vi "Test Evaluate Step A Tolerance Edges.vi"(8 "error in":errorcluster) -> (0 "error out":errorcluster)   [LabVIEW 2026]
doc: "Caraya test of Evaluate Step.vi: settling and the tolerance edges 98.0/102.0 in, 97.999/102.001 out for sp 100 tol 2 (EVS-1..5)."
uses:
  <vilib>/addons/_JKI Toolkits/Caraya/classes/Test/Test.lvclass
  <vilib>/addons/_JKI Toolkits/Caraya/classes/Assert/Assert.lvclass
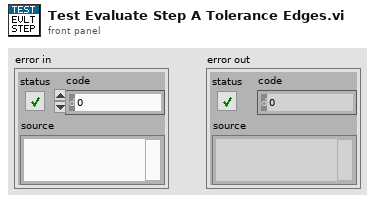
[diagram p1: front panel]
types:
  T1 = cluster{"pressure_bar":dbl, "flow_lpm":dbl, "displacement_mm":dbl, "timestamp_ms":dbl}
  T2 = cluster{"step_no":i32, "step_name":string, "command_type":string, "pressure_sp_bar":dbl, "flow_sp_lpm":dbl, "displacement_sp_mm":dbl, "monitored_io":string, "tolerance_bar":dbl, "dwell_time_ms":i32, "timeout_ms":i32, "expected_result":string}
  T3 = typedef "Step Phase.ctl" = enum16{"Idle", "Settling", "Dwell", "Complete"}
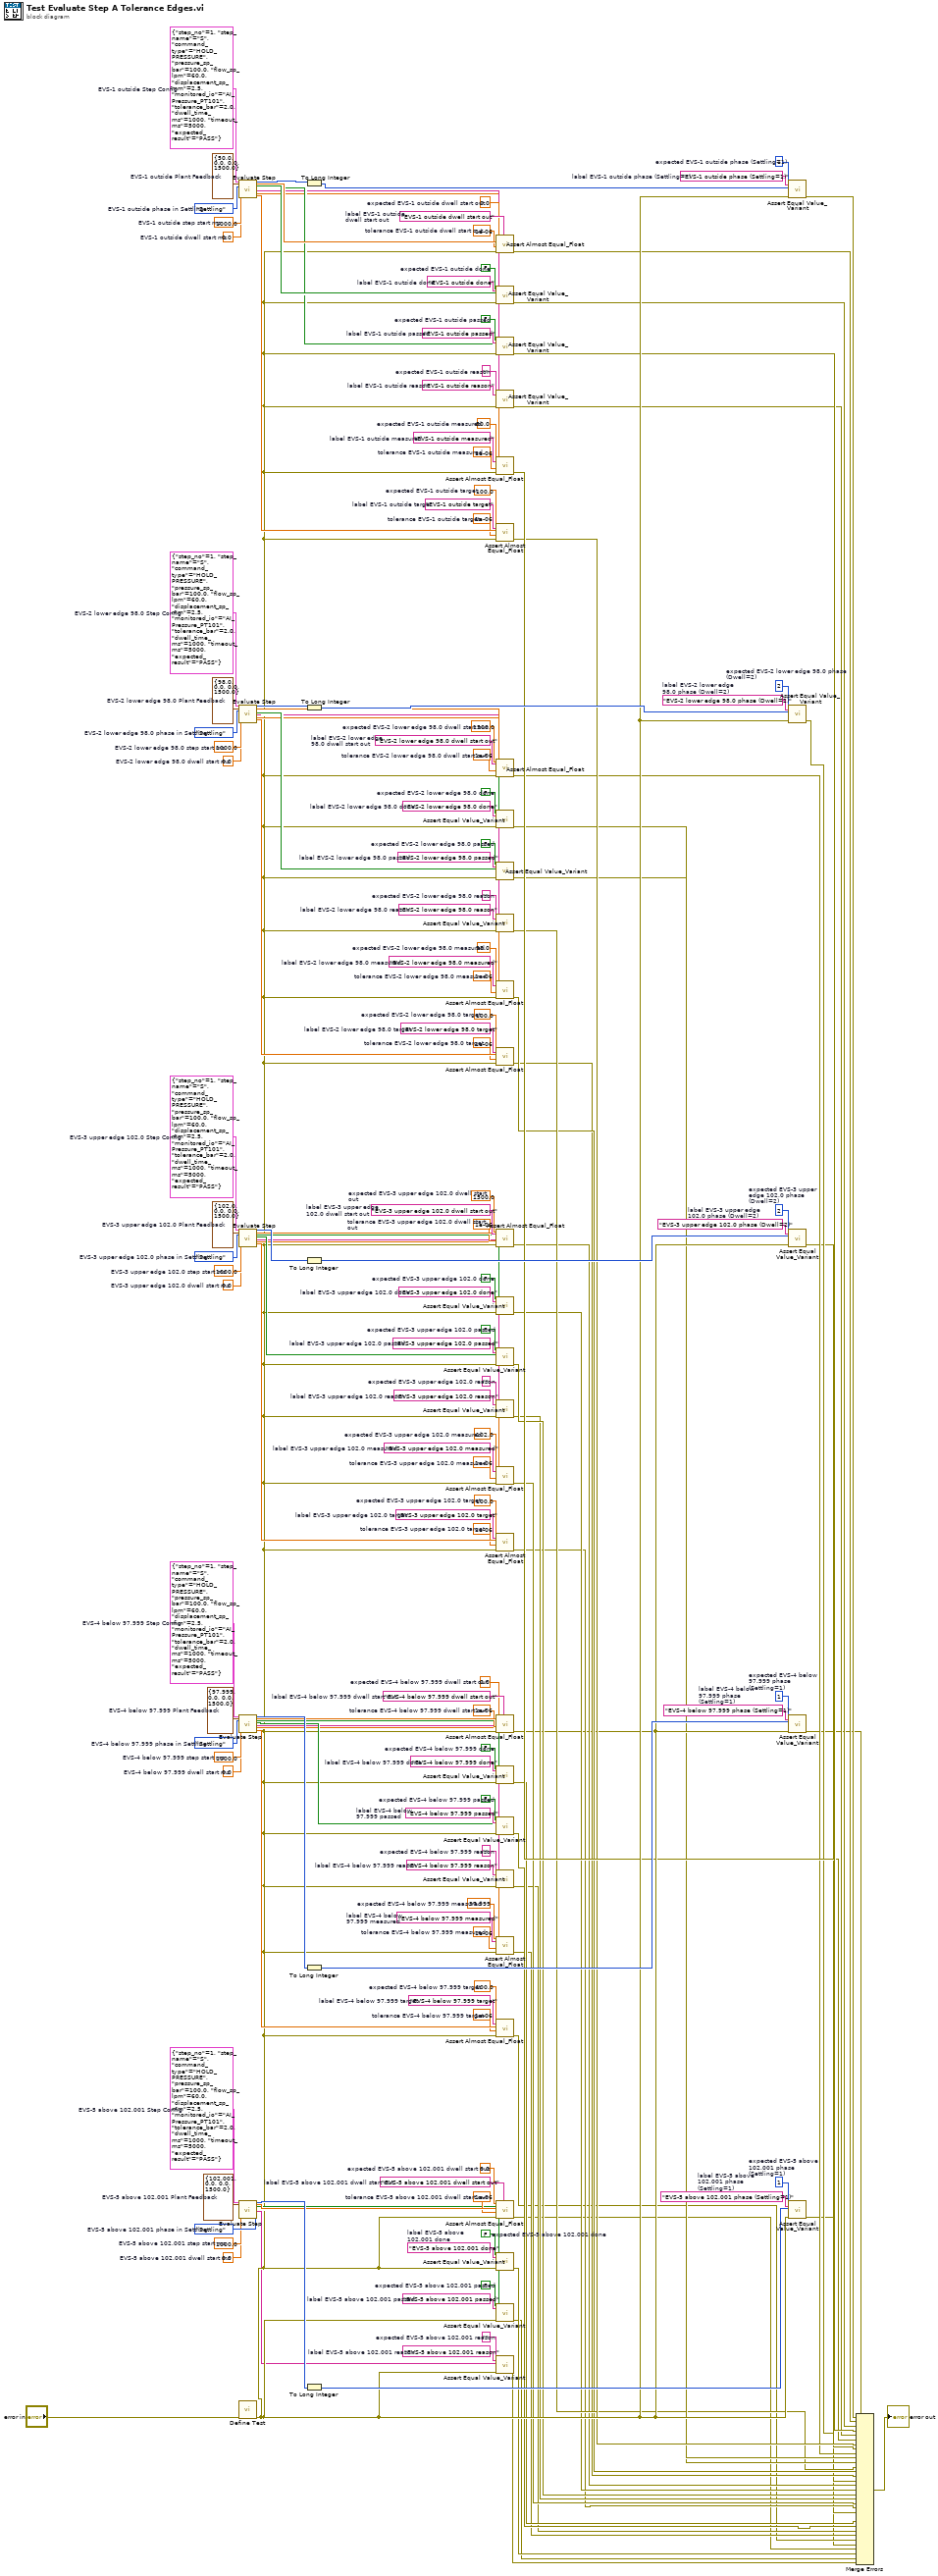
[diagram p0: block diagram]
diagram:
  w38 = "EVS-5 above 102.001 reason"  # label EVS-5 above 102.001 reason
  w36 = ""  # expected EVS-5 above 102.001 reason
  w41 = "EVS-5 above 102.001 passed"  # label EVS-5 above 102.001 passed
  w40 = FALSE  # expected EVS-5 above 102.001 passed
  w44 = "EVS-5 above 102.001 done"  # label EVS-5 above 102.001 done
  w43 = FALSE  # expected EVS-5 above 102.001 done
  w48 = "EVS-5 above 102.001 dwell start out"  # label EVS-5 above 102.001 dwell start out
  w45 = 1e-06  # tolerance EVS-5 above 102.001 dwell start out
  w47 = 0.0  # expected EVS-5 above 102.001 dwell start out
  w51 = "EVS-5 above 102.001 phase (Settling=1)"  # label EVS-5 above 102.001 phase (Settling=1)
  w50 = 1  # expected EVS-5 above 102.001 phase (Settling=1)
  w53 = 0.0  # EVS-5 above 102.001 dwell start ms
  w54 = 1000.0  # EVS-5 above 102.001 step start ms
  w55 = enum16{"Idle", "Settling", "Dwell", "Complete"}."Settling"  # EVS-5 above 102.001 phase in Settling
  w56 = T1 {"pressure_bar"=102.001, "flow_lpm"=0.0, "displacement_mm"=0.0, "timestamp_ms"=1500.0}  # EVS-5 above 102.001 Plant Feedback
  w57 = T2 {"step_no"=1, "step_name"="S", "command_type"="HOLD_PRESSURE", "pressure_sp_bar"=100.0, "flow_sp_lpm"=60.0, "displacement_sp_mm"=2.5, "monitored_io"="AI_Pressure_PT101", "tolerance_bar"=2.0, "dwell_time_ms"=1000, "timeout_ms"=5000, "expected_result"="PASS"}  # EVS-5 above 102.001 Step Config
  w61 = "EVS-4 below 97.999 target"  # label EVS-4 below 97.999 target
  w58 = 1e-06  # tolerance EVS-4 below 97.999 target
  w60 = 100.0  # expected EVS-4 below 97.999 target
  w65 = "EVS-4 below 97.999 measured"  # label EVS-4 below 97.999 measured
  w62 = 1e-06  # tolerance EVS-4 below 97.999 measured
  w64 = 97.999  # expected EVS-4 below 97.999 measured
  w68 = "EVS-4 below 97.999 reason"  # label EVS-4 below 97.999 reason
  w67 = ""  # expected EVS-4 below 97.999 reason
  w71 = "EVS-4 below 97.999 passed"  # label EVS-4 below 97.999 passed
  w70 = FALSE  # expected EVS-4 below 97.999 passed
  w74 = "EVS-4 below 97.999 done"  # label EVS-4 below 97.999 done
  w73 = FALSE  # expected EVS-4 below 97.999 done
  w78 = "EVS-4 below 97.999 dwell start out"  # label EVS-4 below 97.999 dwell start out
  w75 = 1e-06  # tolerance EVS-4 below 97.999 dwell start out
  w77 = 0.0  # expected EVS-4 below 97.999 dwell start out
  w81 = "EVS-4 below 97.999 phase (Settling=1)"  # label EVS-4 below 97.999 phase (Settling=1)
  w80 = 1  # expected EVS-4 below 97.999 phase (Settling=1)
  w83 = 0.0  # EVS-4 below 97.999 dwell start ms
  w84 = 1000.0  # EVS-4 below 97.999 step start ms
  w85 = enum16{"Idle", "Settling", "Dwell", "Complete"}."Settling"  # EVS-4 below 97.999 phase in Settling
  w86 = T1 {"pressure_bar"=97.999, "flow_lpm"=0.0, "displacement_mm"=0.0, "timestamp_ms"=1500.0}  # EVS-4 below 97.999 Plant Feedback
  w87 = T2 {"step_no"=1, "step_name"="S", "command_type"="HOLD_PRESSURE", "pressure_sp_bar"=100.0, "flow_sp_lpm"=60.0, "displacement_sp_mm"=2.5, "monitored_io"="AI_Pressure_PT101", "tolerance_bar"=2.0, "dwell_time_ms"=1000, "timeout_ms"=5000, "expected_result"="PASS"}  # EVS-4 below 97.999 Step Config
  w91 = "EVS-3 upper edge 102.0 target"  # label EVS-3 upper edge 102.0 target
  w88 = 1e-06  # tolerance EVS-3 upper edge 102.0 target
  w90 = 100.0  # expected EVS-3 upper edge 102.0 target
  w95 = "EVS-3 upper edge 102.0 measured"  # label EVS-3 upper edge 102.0 measured
  w92 = 1e-06  # tolerance EVS-3 upper edge 102.0 measured
  w94 = 102.0  # expected EVS-3 upper edge 102.0 measured
  w98 = "EVS-3 upper edge 102.0 reason"  # label EVS-3 upper edge 102.0 reason
  w97 = ""  # expected EVS-3 upper edge 102.0 reason
  w101 = "EVS-3 upper edge 102.0 passed"  # label EVS-3 upper edge 102.0 passed
  w100 = FALSE  # expected EVS-3 upper edge 102.0 passed
  w104 = "EVS-3 upper edge 102.0 done"  # label EVS-3 upper edge 102.0 done
  w103 = FALSE  # expected EVS-3 upper edge 102.0 done
  w108 = "EVS-3 upper edge 102.0 dwell start out"  # label EVS-3 upper edge 102.0 dwell start out
  w105 = 1e-06  # tolerance EVS-3 upper edge 102.0 dwell start out
  w107 = 1500.0  # expected EVS-3 upper edge 102.0 dwell start out
  w111 = "EVS-3 upper edge 102.0 phase (Dwell=2)"  # label EVS-3 upper edge 102.0 phase (Dwell=2)
  w110 = 2  # expected EVS-3 upper edge 102.0 phase (Dwell=2)
  w113 = 0.0  # EVS-3 upper edge 102.0 dwell start ms
  w114 = 1000.0  # EVS-3 upper edge 102.0 step start ms
  w115 = enum16{"Idle", "Settling", "Dwell", "Complete"}."Settling"  # EVS-3 upper edge 102.0 phase in Settling
  w116 = T1 {"pressure_bar"=102.0, "flow_lpm"=0.0, "displacement_mm"=0.0, "timestamp_ms"=1500.0}  # EVS-3 upper edge 102.0 Plant Feedback
  w117 = T2 {"step_no"=1, "step_name"="S", "command_type"="HOLD_PRESSURE", "pressure_sp_bar"=100.0, "flow_sp_lpm"=60.0, "displacement_sp_mm"=2.5, "monitored_io"="AI_Pressure_PT101", "tolerance_bar"=2.0, "dwell_time_ms"=1000, "timeout_ms"=5000, "expected_result"="PASS"}  # EVS-3 upper edge 102.0 Step Config
  w121 = "EVS-2 lower edge 98.0 target"  # label EVS-2 lower edge 98.0 target
  w118 = 1e-06  # tolerance EVS-2 lower edge 98.0 target
  w120 = 100.0  # expected EVS-2 lower edge 98.0 target
  w125 = "EVS-2 lower edge 98.0 measured"  # label EVS-2 lower edge 98.0 measured
  w122 = 1e-06  # tolerance EVS-2 lower edge 98.0 measured
  w124 = 98.0  # expected EVS-2 lower edge 98.0 measured
  w128 = "EVS-2 lower edge 98.0 reason"  # label EVS-2 lower edge 98.0 reason
  w127 = ""  # expected EVS-2 lower edge 98.0 reason
  w131 = "EVS-2 lower edge 98.0 passed"  # label EVS-2 lower edge 98.0 passed
  w130 = FALSE  # expected EVS-2 lower edge 98.0 passed
  w134 = "EVS-2 lower edge 98.0 done"  # label EVS-2 lower edge 98.0 done
  w133 = FALSE  # expected EVS-2 lower edge 98.0 done
  w138 = "EVS-2 lower edge 98.0 dwell start out"  # label EVS-2 lower edge 98.0 dwell start out
  w135 = 1e-06  # tolerance EVS-2 lower edge 98.0 dwell start out
  w137 = 1500.0  # expected EVS-2 lower edge 98.0 dwell start out
  w141 = "EVS-2 lower edge 98.0 phase (Dwell=2)"  # label EVS-2 lower edge 98.0 phase (Dwell=2)
  w140 = 2  # expected EVS-2 lower edge 98.0 phase (Dwell=2)
  w143 = 0.0  # EVS-2 lower edge 98.0 dwell start ms
  w144 = 1000.0  # EVS-2 lower edge 98.0 step start ms
  w145 = enum16{"Idle", "Settling", "Dwell", "Complete"}."Settling"  # EVS-2 lower edge 98.0 phase in Settling
  w146 = T1 {"pressure_bar"=98.0, "flow_lpm"=0.0, "displacement_mm"=0.0, "timestamp_ms"=1500.0}  # EVS-2 lower edge 98.0 Plant Feedback
  w147 = T2 {"step_no"=1, "step_name"="S", "command_type"="HOLD_PRESSURE", "pressure_sp_bar"=100.0, "flow_sp_lpm"=60.0, "displacement_sp_mm"=2.5, "monitored_io"="AI_Pressure_PT101", "tolerance_bar"=2.0, "dwell_time_ms"=1000, "timeout_ms"=5000, "expected_result"="PASS"}  # EVS-2 lower edge 98.0 Step Config
  w151 = "EVS-1 outside target"  # label EVS-1 outside target
  w148 = 1e-06  # tolerance EVS-1 outside target
  w150 = 100.0  # expected EVS-1 outside target
  w155 = "EVS-1 outside measured"  # label EVS-1 outside measured
  w152 = 1e-06  # tolerance EVS-1 outside measured
  w154 = 50.0  # expected EVS-1 outside measured
  w158 = "EVS-1 outside reason"  # label EVS-1 outside reason
  w157 = ""  # expected EVS-1 outside reason
  w161 = "EVS-1 outside passed"  # label EVS-1 outside passed
  w160 = FALSE  # expected EVS-1 outside passed
  w164 = "EVS-1 outside done"  # label EVS-1 outside done
  w163 = FALSE  # expected EVS-1 outside done
  w168 = "EVS-1 outside dwell start out"  # label EVS-1 outside dwell start out
  w165 = 1e-06  # tolerance EVS-1 outside dwell start out
  w167 = 0.0  # expected EVS-1 outside dwell start out
  w171 = "EVS-1 outside phase (Settling=1)"  # label EVS-1 outside phase (Settling=1)
  w170 = 1  # expected EVS-1 outside phase (Settling=1)
  w173 = 0.0  # EVS-1 outside dwell start ms
  w174 = 1000.0  # EVS-1 outside step start ms
  w175 = enum16{"Idle", "Settling", "Dwell", "Complete"}."Settling"  # EVS-1 outside phase in Settling
  w176 = T1 {"pressure_bar"=50.0, "flow_lpm"=0.0, "displacement_mm"=0.0, "timestamp_ms"=1500.0}  # EVS-1 outside Plant Feedback
  w177 = T2 {"step_no"=1, "step_name"="S", "command_type"="HOLD_PRESSURE", "pressure_sp_bar"=100.0, "flow_sp_lpm"=60.0, "displacement_sp_mm"=2.5, "monitored_io"="AI_Pressure_PT101", "tolerance_bar"=2.0, "dwell_time_ms"=1000, "timeout_ms"=5000, "expected_result"="PASS"}  # EVS-1 outside Step Config
  n1 = call "Evaluate Step.vi"("Step Config"=w177, "Plant Feedback"=w176, "Step Phase in"=w175, "step start ms"=w174, "dwell start ms"=w173) -> ("Step Phase out"=w172:T3, "dwell start ms out"=w166:dbl, "done"=w162:bool, "passed"=w159:bool, "reason"=w156:string, "measured"=w153:dbl, "target"=w149:dbl)  [unwired: 16 in]
  n2 = call "Evaluate Step.vi"("Step Config"=w147, "Plant Feedback"=w146, "Step Phase in"=w145, "step start ms"=w144, "dwell start ms"=w143) -> ("Step Phase out"=w142:T3, "dwell start ms out"=w136:dbl, "done"=w132:bool, "passed"=w129:bool, "reason"=w126:string, "measured"=w123:dbl, "target"=w119:dbl)  [unwired: 16 in]
  n3 = call "Evaluate Step.vi"("Step Config"=w117, "Plant Feedback"=w116, "Step Phase in"=w115, "step start ms"=w114, "dwell start ms"=w113) -> ("Step Phase out"=w112:T3, "dwell start ms out"=w106:dbl, "done"=w102:bool, "passed"=w99:bool, "reason"=w96:string, "measured"=w93:dbl, "target"=w89:dbl)  [unwired: 16 in]
  n4 = call "Evaluate Step.vi"("Step Config"=w87, "Plant Feedback"=w86, "Step Phase in"=w85, "step start ms"=w84, "dwell start ms"=w83) -> ("Step Phase out"=w82:T3, "dwell start ms out"=w76:dbl, "done"=w72:bool, "passed"=w69:bool, "reason"=w66:string, "measured"=w63:dbl, "target"=w59:dbl)  [unwired: 16 in]
  n5 = call "Evaluate Step.vi"("Step Config"=w57, "Plant Feedback"=w56, "Step Phase in"=w55, "step start ms"=w54, "dwell start ms"=w53) -> ("Step Phase out"=w52:T3, "dwell start ms out"=w46:dbl, "done"=w42:bool, "passed"=w39:bool, "reason"=w35:string)  [unwired: 16 in, 2 out]
  n6 = call <vilib>:"Define Test.vi"("error in (no error)"="error in") -> ("error out"=w37:errorcluster)  [unwired: 9 in, 1 out]
  n7 = To Long Integer(number=w172) -> (32bit integer=w169:i32)
  n8 = To Long Integer(number=w142) -> (32bit integer=w139:i32)
  n9 = To Long Integer(number=w112) -> (32bit integer=w109:i32)
  n10 = To Long Integer(number=w82) -> (32bit integer=w79:i32)
  n11 = To Long Integer(number=w52) -> (32bit integer=w49:i32)
  n12 = call <vilib>:"Assert Almost Equal_Float.vi"("Label"=w168, "error in (no error)"=w37, "Tolerance"=w165, "Actual"=w166, "Expected"=w167) -> ("error out"=w33:errorcluster)  [unwired: 5 in, 1 out]
  n13 = call <vilib>:"Assert Equal Value_Variant.vi"("Label"=w164, "error in (no error)"=w37, "Actual"=w162, "Expected"=w163) -> ("error out"=w32:errorcluster)  [unwired: 6 in, 1 out]
  n14 = call <vilib>:"Assert Equal Value_Variant.vi"("Label"=w161, "error in (no error)"=w37, "Actual"=w159, "Expected"=w160) -> ("error out"=w31:errorcluster)  [unwired: 6 in, 1 out]
  n15 = call <vilib>:"Assert Equal Value_Variant.vi"("Label"=w158, "error in (no error)"=w37, "Actual"=w156, "Expected"=w157) -> ("error out"=w30:errorcluster)  [unwired: 6 in, 1 out]
  n16 = call <vilib>:"Assert Almost Equal_Float.vi"("Label"=w155, "error in (no error)"=w37, "Tolerance"=w152, "Actual"=w153, "Expected"=w154) -> ("error out"=w29:errorcluster)  [unwired: 5 in, 1 out]
  n17 = call <vilib>:"Assert Almost Equal_Float.vi"("Label"=w151, "error in (no error)"=w37, "Tolerance"=w148, "Actual"=w149, "Expected"=w150) -> ("error out"=w28:errorcluster)  [unwired: 5 in, 1 out]
  n18 = call <vilib>:"Assert Almost Equal_Float.vi"("Label"=w138, "error in (no error)"=w37, "Tolerance"=w135, "Actual"=w136, "Expected"=w137) -> ("error out"=w26:errorcluster)  [unwired: 5 in, 1 out]
  n19 = call <vilib>:"Assert Equal Value_Variant.vi"("Label"=w134, "error in (no error)"=w37, "Actual"=w132, "Expected"=w133) -> ("error out"=w25:errorcluster)  [unwired: 6 in, 1 out]
  n20 = call <vilib>:"Assert Equal Value_Variant.vi"("Label"=w131, "error in (no error)"=w37, "Actual"=w129, "Expected"=w130) -> ("error out"=w24:errorcluster)  [unwired: 6 in, 1 out]
  n21 = call <vilib>:"Assert Equal Value_Variant.vi"("Label"=w128, "error in (no error)"=w37, "Actual"=w126, "Expected"=w127) -> ("error out"=w23:errorcluster)  [unwired: 6 in, 1 out]
  n22 = call <vilib>:"Assert Almost Equal_Float.vi"("Label"=w125, "error in (no error)"=w37, "Tolerance"=w122, "Actual"=w123, "Expected"=w124) -> ("error out"=w22:errorcluster)  [unwired: 5 in, 1 out]
  n23 = call <vilib>:"Assert Almost Equal_Float.vi"("Label"=w121, "error in (no error)"=w37, "Tolerance"=w118, "Actual"=w119, "Expected"=w120) -> ("error out"=w21:errorcluster)  [unwired: 5 in, 1 out]
  n24 = call <vilib>:"Assert Almost Equal_Float.vi"("Label"=w108, "error in (no error)"=w37, "Tolerance"=w105, "Actual"=w106, "Expected"=w107) -> ("error out"=w19:errorcluster)  [unwired: 5 in, 1 out]
  n25 = call <vilib>:"Assert Equal Value_Variant.vi"("Label"=w104, "error in (no error)"=w37, "Actual"=w102, "Expected"=w103) -> ("error out"=w18:errorcluster)  [unwired: 6 in, 1 out]
  n26 = call <vilib>:"Assert Equal Value_Variant.vi"("Label"=w101, "error in (no error)"=w37, "Actual"=w99, "Expected"=w100) -> ("error out"=w17:errorcluster)  [unwired: 6 in, 1 out]
  n27 = call <vilib>:"Assert Equal Value_Variant.vi"("Label"=w98, "error in (no error)"=w37, "Actual"=w96, "Expected"=w97) -> ("error out"=w16:errorcluster)  [unwired: 6 in, 1 out]
  n28 = call <vilib>:"Assert Almost Equal_Float.vi"("Label"=w95, "error in (no error)"=w37, "Tolerance"=w92, "Actual"=w93, "Expected"=w94) -> ("error out"=w15:errorcluster)  [unwired: 5 in, 1 out]
  n29 = call <vilib>:"Assert Almost Equal_Float.vi"("Label"=w91, "error in (no error)"=w37, "Tolerance"=w88, "Actual"=w89, "Expected"=w90) -> ("error out"=w14:errorcluster)  [unwired: 5 in, 1 out]
  n30 = call <vilib>:"Assert Almost Equal_Float.vi"("Label"=w78, "error in (no error)"=w37, "Tolerance"=w75, "Actual"=w76, "Expected"=w77) -> ("error out"=w12:errorcluster)  [unwired: 5 in, 1 out]
  n31 = call <vilib>:"Assert Equal Value_Variant.vi"("Label"=w74, "error in (no error)"=w37, "Actual"=w72, "Expected"=w73) -> ("error out"=w11:errorcluster)  [unwired: 6 in, 1 out]
  n32 = call <vilib>:"Assert Equal Value_Variant.vi"("Label"=w71, "error in (no error)"=w37, "Actual"=w69, "Expected"=w70) -> ("error out"=w10:errorcluster)  [unwired: 6 in, 1 out]
  n33 = call <vilib>:"Assert Equal Value_Variant.vi"("Label"=w68, "error in (no error)"=w37, "Actual"=w66, "Expected"=w67) -> ("error out"=w9:errorcluster)  [unwired: 6 in, 1 out]
  n34 = call <vilib>:"Assert Almost Equal_Float.vi"("Label"=w65, "error in (no error)"=w37, "Tolerance"=w62, "Actual"=w63, "Expected"=w64) -> ("error out"=w8:errorcluster)  [unwired: 5 in, 1 out]
  n35 = call <vilib>:"Assert Almost Equal_Float.vi"("Label"=w61, "error in (no error)"=w37, "Tolerance"=w58, "Actual"=w59, "Expected"=w60) -> ("error out"=w7:errorcluster)  [unwired: 5 in, 1 out]
  n36 = call <vilib>:"Assert Almost Equal_Float.vi"("Label"=w48, "error in (no error)"=w37, "Tolerance"=w45, "Actual"=w46, "Expected"=w47) -> ("error out"=w5:errorcluster)  [unwired: 5 in, 1 out]
  n37 = call <vilib>:"Assert Equal Value_Variant.vi"("Label"=w44, "error in (no error)"=w37, "Actual"=w42, "Expected"=w43) -> ("error out"=w4:errorcluster)  [unwired: 6 in, 1 out]
  n38 = call <vilib>:"Assert Equal Value_Variant.vi"("Label"=w41, "error in (no error)"=w37, "Actual"=w39, "Expected"=w40) -> ("error out"=w3:errorcluster)  [unwired: 6 in, 1 out]
  n39 = call <vilib>:"Assert Equal Value_Variant.vi"("Label"=w38, "error in (no error)"=w37, "Actual"=w35, "Expected"=w36) -> ("error out"=w2:errorcluster)  [unwired: 6 in, 1 out]
  n40 = call <vilib>:"Assert Equal Value_Variant.vi"("Label"=w171, "error in (no error)"=w37, "Actual"=w169, "Expected"=w170) -> ("error out"=w34:errorcluster)  [unwired: 6 in, 1 out]
  n41 = call <vilib>:"Assert Equal Value_Variant.vi"("Label"=w141, "error in (no error)"=w37, "Actual"=w139, "Expected"=w140) -> ("error out"=w27:errorcluster)  [unwired: 6 in, 1 out]
  n42 = call <vilib>:"Assert Equal Value_Variant.vi"("Label"=w111, "error in (no error)"=w37, "Actual"=w109, "Expected"=w110) -> ("error out"=w20:errorcluster)  [unwired: 6 in, 1 out]
  n43 = call <vilib>:"Assert Equal Value_Variant.vi"("Label"=w81, "error in (no error)"=w37, "Actual"=w79, "Expected"=w80) -> ("error out"=w13:errorcluster)  [unwired: 6 in, 1 out]
  n44 = call <vilib>:"Assert Equal Value_Variant.vi"("Label"=w51, "error in (no error)"=w37, "Actual"=w49, "Expected"=w50) -> ("error out"=w6:errorcluster)  [unwired: 6 in, 1 out]
  n45 = Merge Errors(w34, w33, w32, w31, w30, w29, w28, w27, w26, w25, w24, w23, w22, w21, w20, w19, w18, w17, w16, w15, w14, w13, w12, w11, w10, w9, w8, w7, w6, w5, w4, w3, w2) -> (→"error out":errorcluster)
